vi "Create Subscriber Custom Data.vi"(8 "error in (no error)":errorcluster, 10 "New FIFO Instance Config":T1 {"Custom Data" format="%.0x"}, 11 "CIF_Iceoryx_PCAP_Universal in":refnum<class "CIF_Iceoryx_PCAP_Universal.lvclass">) -> (0 "error out":errorcluster, 2 "Custom Data":u8[](array[numeric]), 3 "CIF_Iceoryx_PCAP_Universal out":refnum<class "CIF_Iceoryx_PCAP_Universal.lvclass">)   [LabVIEW 2021, in "CIF_Iceoryx_PCAP_Universal.lvclass"]
uses:
  CIF_Iceoryx_PCAP_Universal.lvclass
  ChannelCommon/typedef/New FIFO Instance Configuration.ctl
  Typedef/Buffer Configuration Data.ctl
  ChannelCommon/ChannelCommon.lvlib
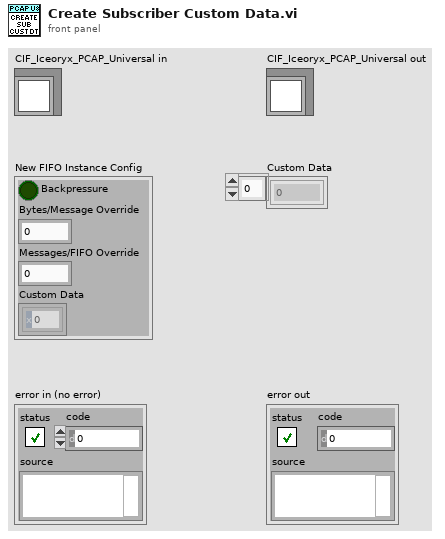
[diagram p1: front panel]
types:
  T1 = typedef "ChannelCommon.lvlib/New FIFO Instance Configuration.ctl" = cluster{"Backpressure":bool, "Bytes/Message Override":u32, "Messages/FIFO Override":u32, "Custom Data":u8[]}
  T2 = typedef "CIF_Iceoryx_PCAP_Universal.lvclass/Buffer Configuration Data.ctl" = cluster{"Backpressure":bool}
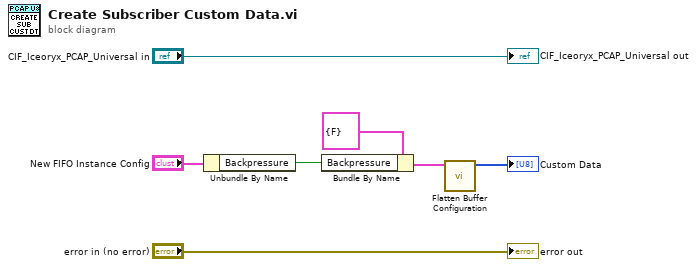
[diagram p0: block diagram]
diagram:
  n1 = Unbundle By Name("New FIFO Instance Config") -> ("Backpressure"=w4:bool)
  n2 = Bundle By Name(cluster=T2 {"Backpressure"=FALSE} ("Buffer Configuration"), "Backpressure"=w4) -> (w3:T2)
  n3 = call "Flatten Buffer Configuration.vi"("Buffer Configuration"=w3) -> ("Flattened Configuration"=→"Custom Data":u8[])  [unwired: 10 in]
  "CIF_Iceoryx_PCAP_Universal out" <- "CIF_Iceoryx_PCAP_Universal in"
  "error out" <- "error in (no error)"
